vi "4Pi Dual DM Control.vi"(7 "Calling VI Ref":refnum<vi>) -> ()   [LabVIEW 2021]
uses:
  4Pi Dual DM - Controls/4Pi Dual DM - Mirror Modes.ctl
  4Pi Dual DM - Controls/DM Max Voltages.ctl
  <vilib>/Utility/miscctls.llb/LVPointTypeDef.ctl
  4Pi Dual DM - Controls/4Pi Dual DM - Mirror Order.ctl
  4Pi Dual DM - Controls/4Pi Dual DM - Standard Action.ctl
  <vilib>/Analysis/baseanly.llb/Mean (DBL).vi
  <vilib>/Utility/file.llb/Read Delimited Spreadsheet (DBL).vi
  <vilib>/Utility/file.llb/Write Delimited Spreadsheet (DBL).vi
  <vilib>/Analysis/NI_AALBase.lvlib
panel:
  in  "DM Max Voltages (V)":T1
  in  "Scan Modes":bool
  in  "Astig On/Off":bool
  in  "Load Astig":bool
  in  "Active Mirror":enum32{"Mirror 1", "Mirror 2"}(radio)
  in  "Clear Modes":bool
  in  "Mirror Modes":T2
  in  "Load Modes":bool
  in  "Save Modes":bool
  in  "Load Flat":bool
  in  "Apply Zero":bool
  in  "Load V Map":bool
  in  "Save V Map":bool
  in  "Apply Flat":bool
  in  "Center Bias":bool
  in  "Quit":bool
  out "Pixel Map (-1 to 1)":dbl[][](graph)
  # "Mode"
  # "Amount (nm)"
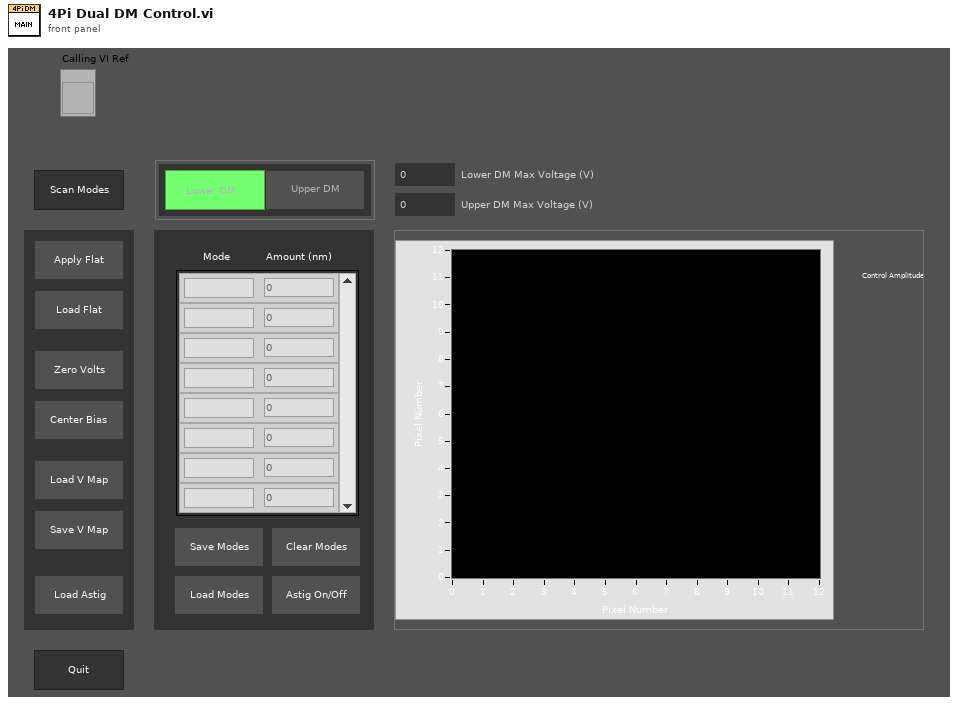
[diagram p1: front panel]
types:
  T1 = typedef "DM Max Voltages.ctl" = cluster{"Lower DM Max Voltage (V)":dbl, "Upper DM Max Voltage (V)":dbl}
  T2 = typedef "4Pi Dual DM - Mirror Modes.ctl" = cluster{"Mode":string, "Amplitude":dbl}[]
  T3 = typedef "4Pi Dual DM - Mirror Order.ctl" = cluster{"Flip Mirror Order":bool}
  T4 = enum16{"Always On", "Always Off", "Off While Running"}
  T5 = typedef "LVPointTypeDef.ctl" = cluster{"Horizontal":i16, "Vertical":i16}
  T6 = typedef "4Pi Dual DM - Standard Action.ctl" = enum16{"Read", "Write"}
  T7 = typedef "LVRectTypeDef.ctl" = cluster{"Left":i16, "Top":i16, "Right":i16, "Bottom":i16}
  T8 = typedef "LVBoundsTypeDef.ctl" = cluster{"Width":u32, "Height":u32}
  T9 = typedef "4Pi Dual DM - Mirror Modes DUAL.ctl" = cluster{"Mode":string, "Amplitude":dbl}[][]
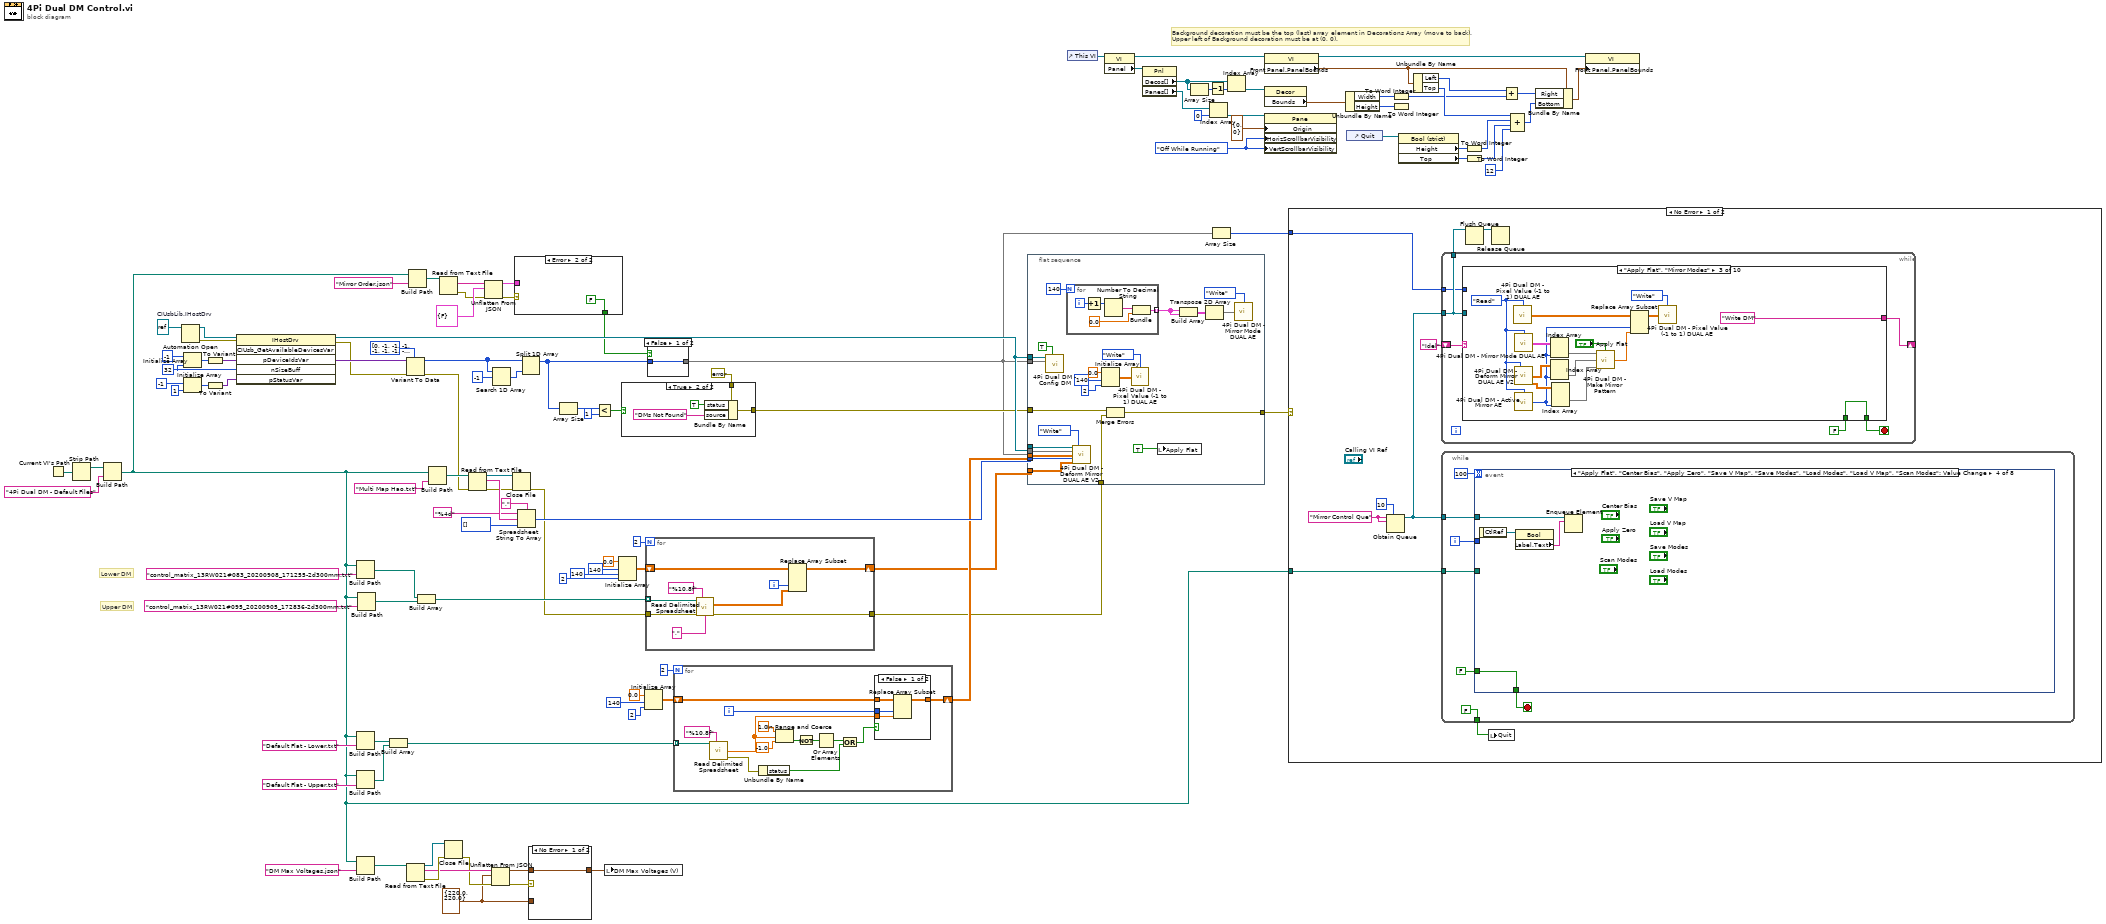
[diagram p0: block diagram]
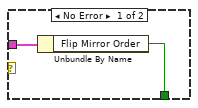
[diagram p2: hidden frame]
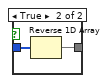
[diagram p4: hidden frame]
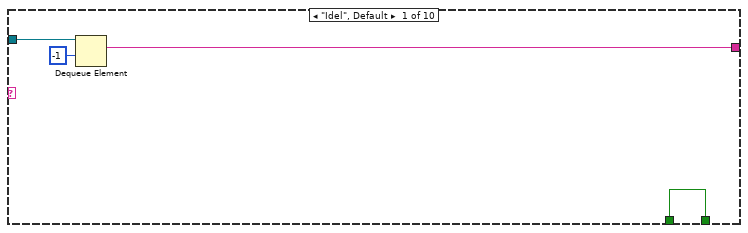
[diagram p5: hidden frame]
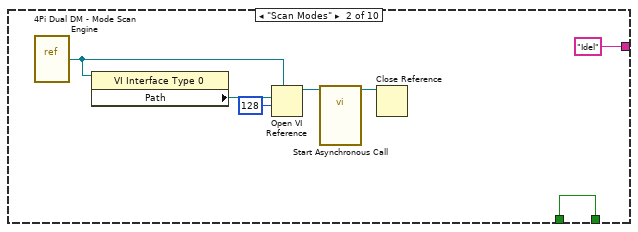
[diagram p6: hidden frame]
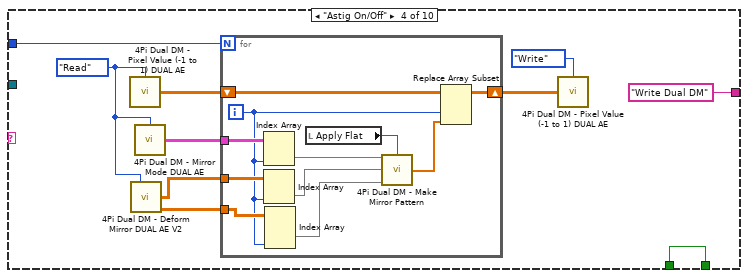
[diagram p7: hidden frame]
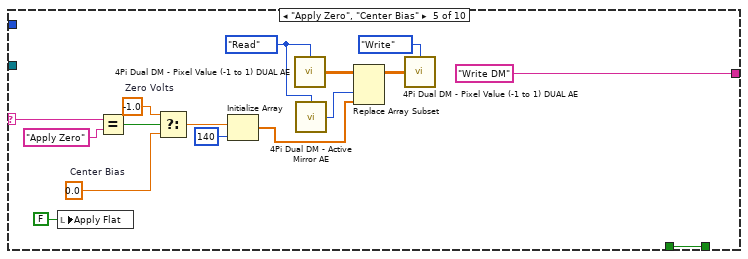
[diagram p8: hidden frame]
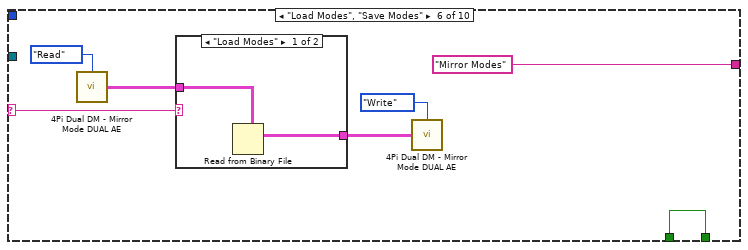
[diagram p9: hidden frame]
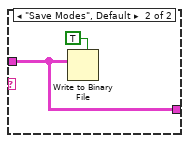
[diagram p10: hidden frame]
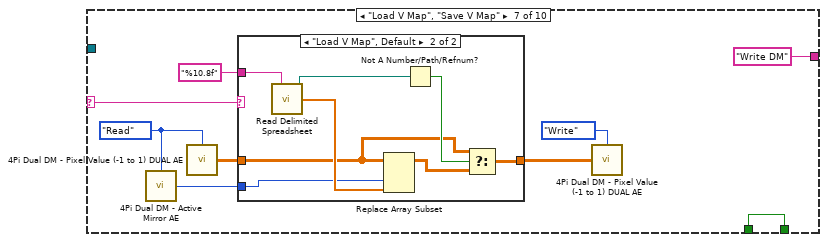
[diagram p11: hidden frame]
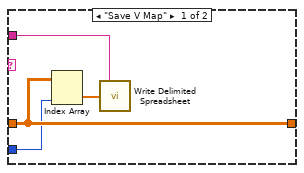
[diagram p12: hidden frame]
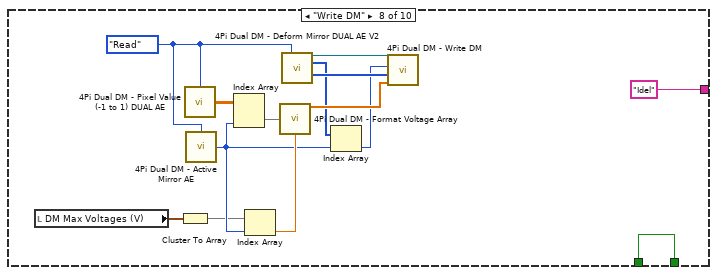
[diagram p13: hidden frame]
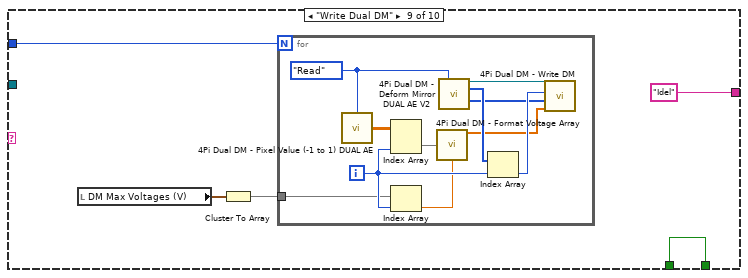
[diagram p14: hidden frame]
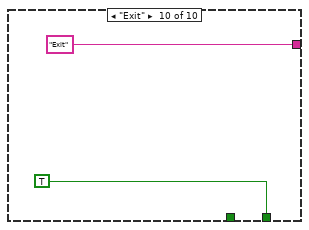
[diagram p15: hidden frame]
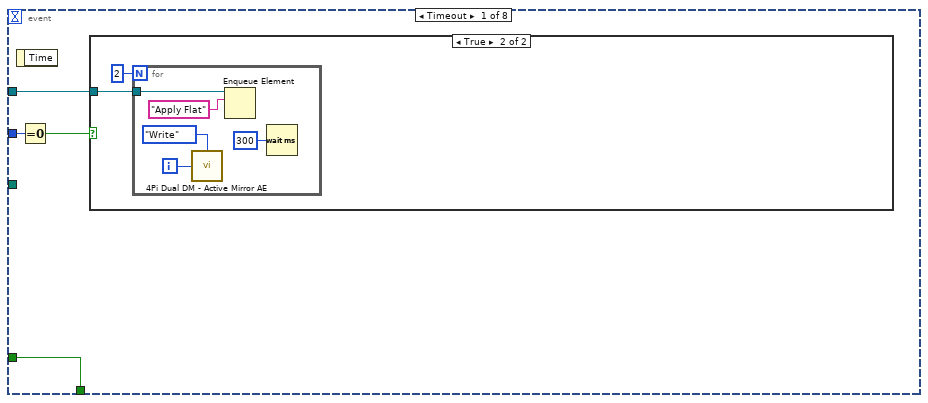
[diagram p16: hidden frame]
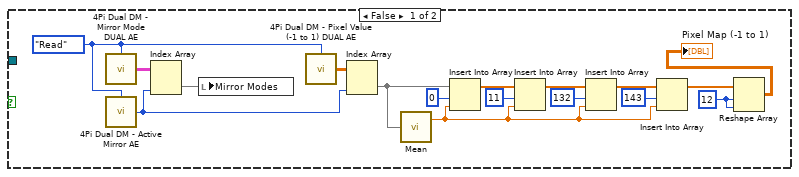
[diagram p17: hidden frame]
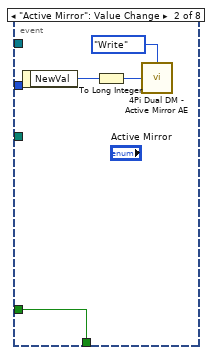
[diagram p18: hidden frame]
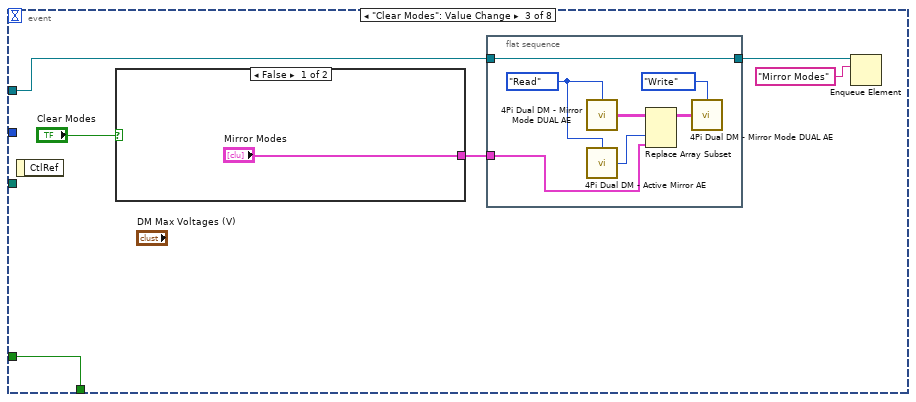
[diagram p19: hidden frame]
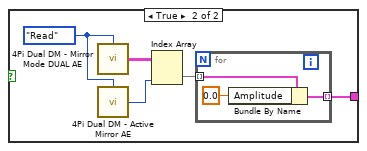
[diagram p20: hidden frame]
diagram:
  w21 = T1 {"Lower DM Max Voltage (V)"=220.0, "Upper DM Max Voltage (V)"=220.0} ("DM Max Voltages (V)")
  w79 = 32 ("dimension size")
  w70 = refnum<k7> refnum  # CIUsbLib.IHostDrv
  w96 = T4."Off While Running" ("Vertical Scrollbar Visibility")
  # "Upper DM"
  # "Lower DM"
  # "Background decoration must be the top (last) array element in Decorations Array (move to back).\nUpper left of Background decoration must be at (0, 0)."
  n1 = Current VI's Path() -> (path=w58:path)
  n2 = Strip Path(path=w58) -> (stripped path=w59:path)  [unwired: 1 out]
  n3 = Build Path(base path=w59, name or relative path="4Pi Dual DM - Default Files") -> (appended path=w10:path)
  n4 = Automation Open(Automation Refnum=w70) -> (Automation Refnum=w75:refnum<k7>, error out=w76:errorcluster)  [unwired: 1 in, 2 out]
  n5 = Initialize Array(-1 ("element"), w79) -> (w72:i32[])
  n6 = Initialize Array(-1 ("element"), 1 ("dimension size")) -> (w71:i32[])
  n7 = To Variant(anything=w72) -> (Variant=w73:variant)
  n8 = To Variant(anything=w71) -> (Variant=w78:variant)
  n9 = invoke class="IHostDrv" method="CIUsb_GetAvailableDevicesVar"(reference=w75, error in=w76, "pDeviceIdsVar"=w73, "nSizeBuff"=w79, "pStatusVar"=w78) -> (reference out=w37:refnum<k7>, error out=w54:errorcluster, "pDeviceIdsVar"=w84:variant)  [unwired: 1 in, 3 out]
  n10 = Build Path(base path=w10, name or relative path="Default Flat - Lower.txt") -> (appended path=w46:path)
  n11 = Build Path(base path=w10, name or relative path="Default Flat - Upper.txt") -> (appended path=w45:path)
  n12 = Build Path(base path=w10, name or relative path="DM Max Voltages.json") -> (appended path=w27:path)
  n13 = Build Path(base path=w10, name or relative path="control_matrix_13RW021#083_20200908_171255-2d300mm.txt") -> (appended path=w8:path)
  n14 = Build Path(base path=w10, name or relative path="control_matrix_13RW021#095_20200905_172836-2d300mm.txt") -> (appended path=w7:path)
  n15 = Build Array(w46, w45) -> (w44:path[])
  n16 = Variant To Data(error in=w54, type=i32[] [0, -1, -1, -1, -1, -1, -1, -1, -1, -1, -1, -1, -1, -1, -1, -1, -1, -1, -1, -1, -1, -1, -1, -1, -1, -1, -1, -1, -1, -1, -1, -1] ("pDeviceIDs"), Variant=w84) -> (data=w82:i32[], error out=w42:errorcluster)
  n17 = Read from Text File(file (use dialog)=w27) -> (refnum out=w26:refnum<file>, text=w24:string, error out=w25:errorcluster)  [unwired: 3 in, 1 out]
  n18 = Build Path(base path=w10, name or relative path="Mirror Order.json") -> (appended path=w34:path)
  n19 = Build Array(w8, w7) -> (w6:path[])
  n20 = Build Path(base path=w10, name or relative path="Multi Map Hao.txt") -> (appended path=w63:path)
  n21 = Read from Text File(file (use dialog)=w34) -> (text=w33:string, error out=w29:errorcluster)  [unwired: 3 in, 2 out]
  n22 = Close File(refnum=w26, error in=w25) -> (error out=w23:errorcluster)  [unwired: 1 out]
  n23 = Read from Text File(file (use dialog)=w63, error in=w42) -> (refnum out=w65:refnum<file>, text=w69:string, error out=w64:errorcluster)  [unwired: 3 out]
  n24 = Unflatten From JSON(JSON string=w33, type and defaults=T3 {"Flip Mirror Order"=FALSE} ("Mirror Order"), error in (no error)=w29) -> (value=w31:T3, error out=w17:errorcluster)  [unwired: 4 in]
  n25 = Unflatten From JSON(JSON string=w24, type and defaults=w21, error in (no error)=w23) -> (value=w20:T1, error out=w22:errorcluster)  [unwired: 4 in]
  n26 = Search 1D Array(1D array=w82, element=-1) -> (index of element=w81:i32)  [unwired: 1 in]
  n27 = Close File(refnum=w65, error in=w64) -> (error out=w4:errorcluster)  [unwired: 1 out]
  n28 = case shown="Error" w17 {
    tunnel: w31 -> [w115 _]
    tunnel: [w114 FALSE ("Flip Mirror Order")] -> w30
    frame No Error {
      n29 = Unbundle By Name(w115) -> ("Flip Mirror Order"=w114:bool)
    }
    frame Error {
    }
  }
  n30 = Spreadsheet String To Array(delimiter (Tab)=",", format string="%4d", spreadsheet string=w69, array type (2D Dbl)=i32[] []) -> (array=w61:i32[])
  n31 = Split 1D Array(array=w82, index=w81) -> (first subarray=w60:i32[])  [unwired: 1 out]
  n32 = case shown="No Error" w22 {
    tunnel: w21 -> [_ w118]
    tunnel: w20 -> [w117 _]
    tunnel: [w117 w118] -> w19
    frame No Error {
    }
    frame Error {
    }
  }
  n33 = Array Size(array=w60) -> (size(s)=w41:i32)
  n34 = Less?(x=w41, y=1) -> (x < y?=w39:bool)
  n35 = local write "DM Max Voltages (V)"(w19) -> ()
  n36 = Initialize Array(0.0 ("element"), 140 ("dimension size"), 140 ("dimension size"), 2 ("dimension size")) -> (w5:dbl[][][])
  n37 = case shown="True" w39 {
    tunnel: [w119 w121] -> w18
    tunnel: errorcluster {"status"=FALSE, "code"=0, "source"=""} ("error out") -> [w119 w120]
    frame False {
    }
    frame True {
      n38 = Bundle By Name(cluster=w120, "status"=TRUE, "source"="DMs Not Found" ("message")) -> (w121:errorcluster)
    }
  }
  n39 = Initialize Array(0.0 ("element"), 140 ("dimension size"), 2 ("dimension size")) -> (w49:dbl[][])
  n40 = for {
    N: 2 -> [_]
    tunnel: w6 -> [w130] mode=indexing
    shift-right: [w128] -> w1
    shift-left: w5 -> [w129]
    tunnel: w4 -> [w125]
    tunnel: [w124] -> w3
    i -> [w127]
    n41 = call-poly <vilib>:"Read Delimited Spreadsheet.vi"("file path (dialog if empty)"=w130, "format (%.3f)"="%10.8f", "error in (no error)"=w125, "delimiter (\\t)"="," ("delimiter (\\t)")) -> ("all rows"=w126:dbl[][], "error out"=w124:errorcluster)  [unwired: 6 in, 4 out]
    n42 = Replace Array Subset(array=w129, new element=w126, index (dim 2)=w127) -> (w128:dbl[][][])  [unwired: 2 in]
  }
  n43 = case shown="False" w30 {
    tunnel: w60 -> [w133 w135]
    tunnel: [w133 w134] -> w16
    frame False {
    }
    frame True {
      n44 = Reverse 1D Array(array=w135) -> (reversed array=w134:i32[])
    }
  }
  n45 = for {
    N: 2 -> [_]
    shift-right: [w146] -> w43
    shift-left: w49 -> [w149]
    tunnel: w44 -> [w140] mode=indexing
    i -> [w148]
    n46 = call-poly <vilib>:"Read Delimited Spreadsheet.vi"("file path (dialog if empty)"=w140, "format (%.3f)"="%10.8f") -> ("first row"=w141:dbl[], "error out"=w139:errorcluster)  [unwired: 8 in, 4 out]
    n47 = Unbundle By Name(w139) -> ("status"=w137:bool)
    n48 = In Range and Coerce(upper limit=1.0, x=w141, lower limit=-1.0) -> (In Range?=w143:bool[])  [unwired: 1 out]
    n49 = Not(x=w143) -> (.not. x?=w144:bool[])
    n50 = Or Array Elements(Boolean array=w144) -> (logical OR=w138:bool)
    n51 = Or(x=w138, y=w137) -> (x .or. y?=w136:bool)
    n52 = case shown="False" w136 {
      tunnel: w149 -> [w153 w154]
      tunnel: w148 -> [w152 _]
      tunnel: [w151 w154] -> w146
      tunnel: w141 -> [w150 _]
      frame False {
        n53 = Replace Array Subset(array=w153, new element=w150, index (col)=w152) -> (w151:dbl[][])  [unwired: 1 in]
      }
      frame True {
      }
    }
  }
  n54 = flat-sequence {
    tunnel: w37 -> [w176]
    tunnel: w61 -> [w174]
    tunnel: w16 -> [w173]
    tunnel: w43 -> [w172]
    tunnel: w18 -> [w171]
    tunnel: w3 -> [w170]
    tunnel: w37 -> [w169]
    tunnel: [w163] -> w36
    tunnel: w16 -> [w162]
    tunnel: w1 -> [w155]
    frame #0 {
      n55 = call "4Pi Dual DM - Config DM.vi"("High Voltage"=TRUE, "Dev IDs"=w173, "Automation Refnum in"=w169) -> ()  [unwired: 7 in, 2 out]
      n56 = for {
        N: 140 -> [_]
        tunnel: [w178] -> w159 mode=indexing
        i -> [w182]
        n57 = Increment(x=w182) -> (x+1=w181:i32)
        n58 = Number To Decimal String(number=w181) -> (decimal integer string=w180:string)  [unwired: 1 in]
        n59 = Bundle(w180, 0.0) -> (w178:cluster{string, dbl})  [unwired: 1 in]
      }
      n60 = call "4Pi Dual DM - Deform Mirror DUAL AE V2.vi"("Refnum In"=w176, "Action"=4Pi_Dual_DM_-_Standard_Action."Write", "IDs In"=w162, "Flat Files In"=w172, "Multi Map Data In"=w174, "Mode Matrix"=w155) -> ()  [unwired: 5 in, 5 out]
      n61 = Initialize Array(0.0 ("element"), 140 ("dimension size"), 2 ("dimension size")) -> (w167:dbl[][])
      n62 = Merge Errors(w171, w170) -> (w163:errorcluster)
      n63 = call "4Pi Dual DM - Pixel Value (-1 to 1) DUAL AE.vi"("Action"=4Pi_Dual_DM_-_Standard_Action."Write", "Pixel Value (-1 to 1)"=w167) -> ()  [unwired: 13 in, 1 out]
      n64 = local write "Apply Flat"(TRUE ("Apply Flat")) -> ()
      n65 = Build Array(w159, w159) -> (w160:cluster{string, dbl}[][])
      n66 = Transpose 2D Array(2D array=w160) -> (transposed array=w161:cluster{string, dbl}[][])
      n67 = call "4Pi Dual DM - Mirror Mode DUAL AE.vi"("Action"=4Pi_Dual_DM_-_Standard_Action."Write", "Mirror Modes In"=w161) -> ()  [unwired: 13 in, 1 out]
    }
  }
  n68 = control-ref of="This VI"() -> (w88:refnum<vi>)
  n69 = property class="VI"(reference=w88) -> (reference out=w97:refnum<vi>, "Panel"=w89:refnum<vi>)  [unwired: 1 in, 1 out]
  n70 = property class="Pnl"(reference=w89) -> ("Decos[]"=w87:refnum<vi>[], "Panes[]"=w93:refnum<vi>[])  [unwired: 1 in, 2 out]
  n71 = Array Size(array=w87) -> (size(s)=w85:i32)
  n72 = Decrement(x=w85) -> (x-1=w86:i32)
  n73 = Index Array(array=w93, index=0) -> (element=w92:refnum<vi>)
  n74 = Array Size(array=w16) -> (size(s)=w15:i32)
  n75 = Index Array(array=w87, index=w86) -> (element=w95:refnum<vi>)
  n76 = property class="VI"(reference=w97) -> (reference out=w99:refnum<vi>, "Front Panel.PanelBounds"=w100:T7)  [unwired: 1 in, 1 out]
  n77 = property class="Decor"(reference=w95) -> ("Bounds"=w98:T8)  [unwired: 1 in, 2 out]
  n78 = property class="Pane"(reference=w92, "Origin"=T5 {"Horizontal"=0, "Vertical"=0}, "HorizScrollbarVisibility"=w96, "VertScrollbarVisibility"=w96) -> ()  [unwired: 1 in, 2 out]
  n79 = case shown="No Error" w36 {
    tunnel: w10 -> [w184 _]
    tunnel: w15 -> [w183 _]
    frame No Error {
      w191 = "Mirror Control Que" ("name (unnamed)")
      n80 = Obtain Queue(max queue size (-1, unlimited)=10, name (unnamed)=w191, element data type=w191) -> (queue out=w186:refnum<queue>)  [unwired: 2 in, 2 out]
      n81 = while {
        tunnel: w186 -> [w193]
        shift-right: [w197] -> _
        shift-left: "Idel" ("name (unnamed)") -> [w196]
        tunnel: [w193] -> w189
        tunnel: w183 -> [w192]
        stop <- w195 stop-if-true
        n82 = case shown="\"Apply Flat\", \"Mirror Modes\"" w196 {
          selector: w196 -> [_ _ _ _ w256 w263 w279 _ _ _]
          tunnel: w193 -> [w201 _ _ _ _ _ _ _ _ _]
          tunnel: [w199 "Idel" ("name (unnamed)") "Write DM" ("name (unnamed)") "Write Dual DM" ("name (unnamed)") "Write DM" ("name (unnamed)") "Mirror Modes" ("name (unnamed)") "Write DM" ("name (unnamed)") "Idel" ("name (unnamed)") "Idel" ("name (unnamed)") "Exit" ("name (unnamed)")] -> w197
          tunnel: [w198 w208 w222 w232 w260 w267 w280 w306 w311 TRUE] -> w195
          tunnel: FALSE -> [w198 w208 w222 w232 w260 w267 w280 w306 w311 _]
          tunnel: w192 -> [_ _ _ w226 _ _ _ _ w307 _]
          frame "Idel", Default {
            n83 = Dequeue Element(queue=w201, timeout in ms (-1)=-1) -> (element=w199:string)  [unwired: 1 in, 3 out]
          }
          frame "Scan Modes" {
            n84 = vi-ref "4Pi Dual DM - Mode Scan Engine.vi"() -> (w202:refnum<vi>)
            n85 = property class="VI Interface Type 0"(reference=w202) -> ("Path"=w203:path)  [unwired: 1 in, 2 out]
            n86 = Open VI Reference(type specifier VI Refnum (for type only)=w202, vi path=w203, options=128) -> (vi reference=w205:refnum<vi>)  [unwired: 3 in, 1 out]
            n87 = call-by-ref "Start Asynchronous Call"(reference=w205) -> (reference out=w206:refnum<vi>)  [unwired: 17 in, 1 out]
            n88 = Close Reference(reference=w206) -> ()  [unwired: 1 in, 1 out]
          }
          frame "Apply Flat", "Mirror Modes" {
            w218 = 4Pi_Dual_DM_-_Standard_Action."Read" ("Action")
            n89 = call "4Pi Dual DM - Pixel Value (-1 to 1) DUAL AE.vi"("Action"=w218) -> ("Pixel Value (-1 to 1) Out"=w219:dbl[][])  [unwired: 14 in]
            n90 = call "4Pi Dual DM - Mirror Mode DUAL AE.vi"("Action"=w218) -> ("Mirror Modes Out"=w215:T9)  [unwired: 14 in]
            n91 = call "4Pi Dual DM - Deform Mirror DUAL AE V2.vi"("Action"=w218) -> ("Flat Files Out"=w213:dbl[][], "Mode Matrix Out"=w211:dbl[][][])  [unwired: 10 in, 3 out]
            n92 = call "4Pi Dual DM - Active Mirror AE.vi"("Action"=w218) -> ("Active Mirror"=w210:i32)  [unwired: 14 in]
            n93 = Index Array(array=w215, index (col)=w210) -> (element=w216:cluster{"Mode":string, "Amplitude":dbl}[])  [unwired: 1 in]
            n94 = Index Array(array=w213, index (col)=w210) -> (element=w214:dbl[])  [unwired: 1 in]
            n95 = Index Array(array=w211, index (dim 2)=w210) -> (element=w209:dbl[][])  [unwired: 2 in]
            n96 = call "4Pi Dual DM - Make Mirror Pattern.vi"("Mirror Modes In"=w216, "Flat On?"="Apply Flat", "Flat File In"=w214, "Mirror Modes Array"=w209) -> ("Pixel Value U (-1 to 1)"=w220:dbl[])  [unwired: 11 in]
            n97 = Replace Array Subset(array=w219, new element=w220, index (col)=w210) -> (w221:dbl[][])  [unwired: 1 in]
            n98 = call "4Pi Dual DM - Pixel Value (-1 to 1) DUAL AE.vi"("Action"=4Pi_Dual_DM_-_Standard_Action."Write", "Pixel Value (-1 to 1)"=w221) -> ()  [unwired: 13 in, 1 out]
          }
          frame "Astig On/Off" {
            w231 = 4Pi_Dual_DM_-_Standard_Action."Read" ("Action")
            n99 = call "4Pi Dual DM - Pixel Value (-1 to 1) DUAL AE.vi"("Action"=w231) -> ("Pixel Value (-1 to 1) Out"=w230:dbl[][])  [unwired: 14 in]
            n100 = call "4Pi Dual DM - Deform Mirror DUAL AE V2.vi"("Action"=w231) -> ("Flat Files Out"=w228:dbl[][], "Mode Matrix Out"=w227:dbl[][][])  [unwired: 10 in, 3 out]
            n101 = call "4Pi Dual DM - Mirror Mode DUAL AE.vi"("Action"=w231) -> ("Mirror Modes Out"=w229:T9)  [unwired: 14 in]
            n102 = for {
              N: w226 -> [_]
              tunnel: w229 -> [w239]
              tunnel: w228 -> [w238]
              tunnel: w227 -> [w236]
              shift-right: [w237] -> w224
              shift-left: w230 -> [w240]
              i -> [w235]
              n103 = Index Array(array=w239, index (col)=w235) -> (element=w243:cluster{"Mode":string, "Amplitude":dbl}[])  [unwired: 1 in]
              n104 = Index Array(array=w238, index (col)=w235) -> (element=w244:dbl[])  [unwired: 1 in]
              n105 = Index Array(array=w236, index (dim 2)=w235) -> (element=w234:dbl[][])  [unwired: 2 in]
              n106 = local read "Apply Flat"() -> (w241:bool)
              n107 = call "4Pi Dual DM - Make Mirror Pattern.vi"("Mirror Modes In"=w243, "Flat On?"=w241, "Flat File In"=w244, "Mirror Modes Array"=w234) -> ("Pixel Value U (-1 to 1)"=w242:dbl[])  [unwired: 11 in]
              n108 = Replace Array Subset(array=w240, new element=w242, index (col)=w235) -> (w237:dbl[][])  [unwired: 1 in]
            }
            n109 = call "4Pi Dual DM - Pixel Value (-1 to 1) DUAL AE.vi"("Action"=4Pi_Dual_DM_-_Standard_Action."Write", "Pixel Value (-1 to 1)"=w224) -> ()  [unwired: 13 in, 1 out]
          }
          frame "Apply Zero", "Center Bias" {
            w248 = 4Pi_Dual_DM_-_Standard_Action."Read" ("Action")
            w252 = -1.0  # Zero Volts
            w254 = 0.0  # Center Bias
            n110 = local write "Apply Flat"(FALSE ("Apply Flat")) -> ()
            n111 = Equal?(x=w256, y="Apply Zero") -> (x = y?=w255:bool)
            n112 = Select(t=w252, s=w255, f=w254) -> (s? t:f=w253:dbl)
            n113 = Initialize Array(w253, 140 ("dimension size")) -> (w245:dbl[])
            n114 = call "4Pi Dual DM - Pixel Value (-1 to 1) DUAL AE.vi"("Action"=w248) -> ("Pixel Value (-1 to 1) Out"=w246:dbl[][])  [unwired: 14 in]
            n115 = call "4Pi Dual DM - Active Mirror AE.vi"("Action"=w248) -> ("Active Mirror"=w247:i32)  [unwired: 14 in]
            n116 = Replace Array Subset(array=w246, new element=w245, index (col)=w247) -> (w250:dbl[][])  [unwired: 1 in]
            n117 = call "4Pi Dual DM - Pixel Value (-1 to 1) DUAL AE.vi"("Action"=4Pi_Dual_DM_-_Standard_Action."Write", "Pixel Value (-1 to 1)"=w250) -> ()  [unwired: 13 in, 1 out]
          }
          frame "Load Modes", "Save Modes" {
            n118 = call "4Pi Dual DM - Mirror Mode DUAL AE.vi"("Action"=4Pi_Dual_DM_-_Standard_Action."Read") -> ("Mirror Modes Out"=w262:T9)  [unwired: 14 in]
            n119 = case shown="\"Load Modes\"" w263 {
              tunnel: w262 -> [w269 w270]
              tunnel: [w268 w270] -> w261
              frame "Load Modes" {
                n120 = Read from Binary File(5:w269) -> (2:w268:T9)  [unwired: 5 in, 3 out]
              }
              frame "Save Modes", Default {
                n121 = Write to Binary File(data=w270, 5:TRUE ("prepend array or string size? (T)")) -> ()  [unwired: 4 in, 3 out]
              }
            }
            n122 = call "4Pi Dual DM - Mirror Mode DUAL AE.vi"("Action"=4Pi_Dual_DM_-_Standard_Action."Write", "Mirror Modes In"=w261) -> ()  [unwired: 13 in, 1 out]
          }
          frame "Load V Map", "Save V Map" {
            w273 = 4Pi_Dual_DM_-_Standard_Action."Read" ("Action")
            n123 = call "4Pi Dual DM - Active Mirror AE.vi"("Action"=w273) -> ("Active Mirror"=w272:i32)  [unwired: 14 in]
            n124 = call "4Pi Dual DM - Pixel Value (-1 to 1) DUAL AE.vi"("Action"=w273) -> ("Pixel Value (-1 to 1) Out"=w277:dbl[][])  [unwired: 14 in]
            n125 = case shown="\"Load V Map\", Default" w279 {
              tunnel: w277 -> [w283 w285]
              tunnel: "%10.8f" -> [w284 w292]
              tunnel: [w283 w289] -> w274
              tunnel: w272 -> [w281 w286]
              frame "Save V Map" {
                n126 = Index Array(array=w283, index (col)=w281) -> (element=w282:dbl[])  [unwired: 1 in]
                n127 = call-poly <vilib>:"Write Delimited Spreadsheet.vi"("format (%.3f)"=w284, "1D data"=w282) -> ()  [unwired: 12 in, 2 out]
              }
              frame "Load V Map", Default {
                n128 = call-poly <vilib>:"Read Delimited Spreadsheet.vi"("format (%.3f)"=w292) -> ("new file path (Not A Path if cancelled)"=w291:path, "first row"=w287:dbl[])  [unwired: 9 in, 4 out]
                n129 = Replace Array Subset(array=w285, new element=w287, index (col)=w286) -> (w288:dbl[][])  [unwired: 1 in]
                n130 = Not A Number/Path/Refnum?(number/path/refnum=w291) -> (NaN/Path/Refnum?=w290:bool)
                n131 = Select(t=w285, s=w290, f=w288) -> (s? t:f=w289:dbl[][])
              }
            }
            n132 = call "4Pi Dual DM - Pixel Value (-1 to 1) DUAL AE.vi"("Action"=4Pi_Dual_DM_-_Standard_Action."Write", "Pixel Value (-1 to 1)"=w274) -> ()  [unwired: 13 in, 1 out]
          }
          frame "Write DM" {
            w299 = 4Pi_Dual_DM_-_Standard_Action."Read" ("Action")
            n133 = local read "DM Max Voltages (V)"() -> (w294:T1)
            n134 = Cluster To Array(cluster=w294) -> (array=w293:dbl[])
            n135 = call "4Pi Dual DM - Pixel Value (-1 to 1) DUAL AE.vi"("Action"=w299) -> ("Pixel Value (-1 to 1) Out"=w301:dbl[][])  [unwired: 14 in]
            n136 = call "4Pi Dual DM - Active Mirror AE.vi"("Action"=w299) -> ("Active Mirror"=w295:i32)  [unwired: 14 in]
            n137 = Index Array(array=w301, index (col)=w295) -> (element=w300:dbl[])  [unwired: 1 in]
            n138 = Index Array(array=w293, index=w295) -> (element=w296:dbl)
            n139 = call "4Pi Dual DM - Format Voltage Array.vi"("Pixel Level (-1 to 1)"=w300, "Max DM Voltage"=w296) -> ("Voltage Array (Volts)"=w302:dbl[])  [unwired: 12 in, 1 out]
            n140 = call "4Pi Dual DM - Deform Mirror DUAL AE V2.vi"("Action"=w299) -> ("Refnum Out"=w304:refnum<k7>, "IDs Out"=w298:i32[], "Multi Map Data Out"=w303:i32[])  [unwired: 10 in, 2 out]
            n141 = Index Array(array=w298, index=w295) -> (element=w297:i32)
            n142 = call "4Pi Dual DM - Write DM.vi"("reference in"=w304, "nDevId"=w297, "MultiDM  Mapping"=w303, "Voltage Array in"=w302) -> ()  [unwired: 2 in, 2 out]
          }
          frame "Write Dual DM" {
            n143 = local read "DM Max Voltages (V)"() -> (w309:T1)
            n144 = Cluster To Array(cluster=w309) -> (array=w308:dbl[])
            n145 = for {
              N: w307 -> [_]
              tunnel: w308 -> [w313]
              i -> [w314]
              w320 = 4Pi_Dual_DM_-_Standard_Action."Read" ("Action")
              n146 = call "4Pi Dual DM - Pixel Value (-1 to 1) DUAL AE.vi"("Action"=w320) -> ("Pixel Value (-1 to 1) Out"=w318:dbl[][])  [unwired: 14 in]
              n147 = Index Array(array=w318, index (col)=w314) -> (element=w319:dbl[])  [unwired: 1 in]
              n148 = Index Array(array=w313, index=w314) -> (element=w312:dbl)
              n149 = call "4Pi Dual DM - Format Voltage Array.vi"("Pixel Level (-1 to 1)"=w319, "Max DM Voltage"=w312) -> ("Voltage Array (Volts)"=w317:dbl[])  [unwired: 12 in, 1 out]
              n150 = call "4Pi Dual DM - Deform Mirror DUAL AE V2.vi"("Action"=w320) -> ("Refnum Out"=w315:refnum<k7>, "IDs Out"=w321:i32[], "Multi Map Data Out"=w316:i32[])  [unwired: 10 in, 2 out]
              n151 = Index Array(array=w321, index=w314) -> (element=w322:i32)
              n152 = call "4Pi Dual DM - Write DM.vi"("reference in"=w315, "nDevId"=w322, "MultiDM  Mapping"=w316, "Voltage Array in"=w317) -> ()  [unwired: 2 in, 2 out]
            }
          }
          frame "Exit" {
          }
        }
      }
      n153 = while {
        tunnel: w186 -> [w327]
        tunnel: [FALSE] -> w185
        tunnel: w184 -> [w325]
        i -> [w328]
        stop <- w331 stop-if-true
        n154 = event shown="[3] \"Apply Flat\", \"Center Bias\", \"Apply Zero\", \"Save V Map\", \"Save Modes\", \"Load Modes\", \"Load V Map\", \"Scan Modes\": Value Change" {
          selector: _ -> [_ _ _ _ _ _ _ _]
          dyn-events: _ -> [_ _ _ _ _ _ _ _]
          timeout: 100 -> [_ _ _ _ _ _ _ _]
          tunnel: [w335 w363 w369 w389 w394 w418 w427 w456] -> w331
          tunnel: FALSE -> [w335 w363 w369 w389 w394 w418 w427 _]
          tunnel: w328 -> [w334 _ _ _ _ _ _ _]
          tunnel: w327 -> [w332 _ w368 w388 _ _ w424 w454]
          tunnel: w325 -> [_ _ _ _ w393 w416 _ _]
          event Timeout {
            n155 = event-data() -> ()  [unwired: 1 in, 1 out]
            n156 = Equal To 0?(x=w334) -> (x = 0?=w333:bool)
            n157 = case shown="True" w333 {
              tunnel: w332 -> [_ w354]
              frame False {
                w348 = 12 ("dimension size")
                w349 = 4Pi_Dual_DM_-_Standard_Action."Read" ("Action")
                n158 = call "4Pi Dual DM - Mirror Mode DUAL AE.vi"("Action"=w349) -> ("Mirror Modes Out"=w336:T9)  [unwired: 14 in]
                n159 = call "4Pi Dual DM - Active Mirror AE.vi"("Action"=w349) -> ("Active Mirror"=w351:i32)  [unwired: 14 in]
                n160 = Index Array(array=w336, index (col)=w351) -> (element=w337:cluster{"Mode":string, "Amplitude":dbl}[])  [unwired: 1 in]
                n161 = local write "Mirror Modes"(w337) -> ()
                n162 = call "4Pi Dual DM - Pixel Value (-1 to 1) DUAL AE.vi"("Action"=w349) -> ("Pixel Value (-1 to 1) Out"=w350:dbl[][])  [unwired: 14 in]
                n163 = Index Array(array=w350, index (col)=w351) -> (element=w352:dbl[])  [unwired: 1 in]
                n164 = call-poly <vilib>:"Mean.vi"("X"=w352) -> ("mean"=w346:dbl)  [unwired: 1 out]
                n165 = Insert Into Array(array=w352, index=0, new element=w346) -> (w341:dbl[])
                n166 = Insert Into Array(array=w341, index=11, new element=w346) -> (w343:dbl[])
                n167 = Insert Into Array(array=w343, index=132, new element=w346) -> (w345:dbl[])
                n168 = Insert Into Array(array=w345, index=143, new element=w346) -> (w338:dbl[])
                n169 = Reshape Array(w338, w348, w348) -> (→"Pixel Map (-1 to 1)":dbl[][])
              }
              frame True {
                n170 = for {
                  N: 2 -> [_]
                  tunnel: w354 -> [w359]
                  i -> [w355]
                  n171 = call "4Pi Dual DM - Active Mirror AE.vi"("Action"=4Pi_Dual_DM_-_Standard_Action."Write", "Active Mirror In"=w355) -> ()  [unwired: 13 in, 1 out]
                  n172 = Enqueue Element(queue=w359, element="Apply Flat") -> ()  [unwired: 2 in, 3 out]
                  n173 = Wait (ms)(milliseconds to wait=u32 300) -> ()  [unwired: 1 out]
                }
              }
            }
          }
          event "Active Mirror": Value Change {
            n174 = event-data() -> ("NewVal"=w362:enum32{"Mirror 1", "Mirror 2"})  [unwired: 1 in]
            n175 = To Long Integer(number=w362) -> (32bit integer=w361:i32)
            n176 = call "4Pi Dual DM - Active Mirror AE.vi"("Action"=4Pi_Dual_DM_-_Standard_Action."Write", "Active Mirror In"=w361) -> ()  [unwired: 13 in, 1 out]
          }
          event "Clear Modes": Value Change {
            n177 = event-data() -> ()  [unwired: 1 in, 1 out]
            n178 = case shown="False" "Clear Modes" {
              tunnel: ["Mirror Modes" w371] -> w364
              frame False {
              }
              frame True {
                w374 = 4Pi_Dual_DM_-_Standard_Action."Read" ("Action")
                n179 = call "4Pi Dual DM - Mirror Mode DUAL AE.vi"("Action"=w374) -> ("Mirror Modes Out"=w373:T9)  [unwired: 14 in]
                n180 = call "4Pi Dual DM - Active Mirror AE.vi"("Action"=w374) -> ("Active Mirror"=w375:i32)  [unwired: 14 in]
                n181 = Index Array(array=w373, index (col)=w375) -> (element=w372:cluster{"Mode":string, "Amplitude":dbl}[])  [unwired: 1 in]
                n182 = for {
                  tunnel: w372 -> [w378] mode=indexing
                  tunnel: [w376] -> w371 mode=indexing
                  n183 = Bundle By Name(cluster=w378, "Amplitude"=0.0) -> (w376:cluster{"Mode":string, "Amplitude":dbl})
                }
              }
            }
            n184 = flat-sequence {
              tunnel: w364 -> [w379]
              tunnel: w368 -> [w385]
              tunnel: [w385] -> w366
              frame #0 {
                w382 = 4Pi_Dual_DM_-_Standard_Action."Read" ("Action")
                n185 = call "4Pi Dual DM - Mirror Mode DUAL AE.vi"("Action"=w382) -> ("Mirror Modes Out"=w381:T9)  [unwired: 14 in]
                n186 = call "4Pi Dual DM - Active Mirror AE.vi"("Action"=w382) -> ("Active Mirror"=w383:i32)  [unwired: 14 in]
                n187 = Replace Array Subset(array=w381, new element=w379, index (col)=w383) -> (w384:T9)  [unwired: 1 in]
                n188 = call "4Pi Dual DM - Mirror Mode DUAL AE.vi"("Action"=4Pi_Dual_DM_-_Standard_Action."Write", "Mirror Modes In"=w384) -> ()  [unwired: 13 in, 1 out]
              }
            }
            n189 = Enqueue Element(queue=w366, element="Mirror Modes") -> ()  [unwired: 2 in, 3 out]
          }
          event "Apply Flat", "Center Bias", "Apply Zero", "Save V Map", "Save Modes", "Load Modes", "Load V Map", "Scan Modes": Value Change {
            n190 = event-data() -> ("CtlRef"=w387:refnum<vi>)  [unwired: 1 in]
            n191 = property class="Bool"(reference=w387) -> ("Label.Text"=w386:string)  [unwired: 1 in, 2 out]
            n192 = Enqueue Element(queue=w388, element=w386) -> ()  [unwired: 2 in, 3 out]
          }
          event "Load Flat": Value Change {
            n193 = event-data() -> ()  [unwired: 1 in, 1 out]
            n194 = call "File Dialog"("start path"=w393, "prompt"="Select Flat File") -> ("selected path"=w390:path, "error out"=w391:errorcluster)  [unwired: 10 in, 2 out]
            n195 = case shown="No Error" w391 {
              tunnel: w390 -> [w395 _]
              frame No Error {
                w402 = 4Pi_Dual_DM_-_Standard_Action."Read" ("Action")
                n196 = call-poly <vilib>:"Read Delimited Spreadsheet.vi"("file path (dialog if empty)"=w395, "format (%.3f)"="%10.8f") -> ("first row"=w411:dbl[])  [unwired: 8 in, 5 out]
                n197 = In Range and Coerce(upper limit=1.0, x=w411, lower limit=-1.0) -> (coerced(x)=w396:dbl[], In Range?=w408:bool[])
                n198 = call "4Pi Dual DM - Deform Mirror DUAL AE V2.vi"("Action"=w402) -> ("Refnum Out"=w397:refnum<k7>, "IDs Out"=w398:i32[], "Flat Files Out"=w403:dbl[][], "Multi Map Data Out"=w399:i32[], "Mode Matrix Out"=w400:dbl[][][])  [unwired: 10 in]
                n199 = call "4Pi Dual DM - Active Mirror AE.vi"("Action"=w402) -> ("Active Mirror"=w405:i32)  [unwired: 14 in]
                n200 = Not(x=w408) -> (.not. x?=w407:bool[])
                n201 = Replace Array Subset(array=w403, new element=w396, index (col)=w405) -> (w404:dbl[][])  [unwired: 1 in]
                n202 = Or Array Elements(Boolean array=w407) -> (logical OR=w406:bool)
                n203 = call "4Pi Dual DM - Deform Mirror DUAL AE V2.vi"("Refnum In"=w397, "Action"=4Pi_Dual_DM_-_Standard_Action."Write", "IDs In"=w398, "Flat Files In"=w404, "Multi Map Data In"=w399, "Mode Matrix"=w400) -> ()  [unwired: 5 in, 5 out]
                n204 = case shown="True" w406 {
                  frame False {
                  }
                  frame True {
                    n205 = One Button Dialog(message="Flat File Out of Range [-1, 1]") -> ()  [unwired: 1 in, 1 out]
                  }
                }
              }
              frame Error {
              }
            }
          }
          event "Load Astig": Value Change {
            n206 = event-data() -> ()  [unwired: 1 in, 1 out]
            n207 = call "File Dialog2"("start path"=w416, "prompt"="Select Astigmatism File") -> ("selected path"=w414:path, "error out"=w415:errorcluster)  [unwired: 10 in, 2 out]
            n208 = case shown="No Error" w415 {
              tunnel: w414 -> [w419 _]
              frame No Error {
                n209 = call "4Pi Dual DM - Astig Modes AE.vi"("Action"=4Pi_Dual_DM_-_Standard_Action."Read") -> ("Mirror Modes Out"=w423:T9)  [unwired: 14 in]
                n210 = Read from Binary File(5:w423, 11:w419) -> (2:w420:T9)  [unwired: 4 in, 3 out]
                n211 = call "4Pi Dual DM - Astig Modes AE.vi"("Action"=4Pi_Dual_DM_-_Standard_Action."Write", "Mirror Modes In"=w420) -> ()  [unwired: 13 in, 1 out]
              }
              frame Error {
              }
            }
          }
          event "Astig On/Off": Value Change {
            n212 = event-data() -> ()  [unwired: 1 in, 1 out]
            n213 = case shown="True" "Astig On/Off" {
              tunnel: [w432 w444] -> w425
              frame False {
                n214 = for {
                  N: 2 -> [_]
                  tunnel: [w435] -> w433 mode=indexing
                  i -> [w436]
                  n215 = call "4Pi Dual DM - Mirror Mode DUAL AE.vi"("Action"=4Pi_Dual_DM_-_Standard_Action."Read") -> ("Mirror Modes Out"=w438:T9)  [unwired: 14 in]
                  n216 = Index Array(array=w438, index (col)=w436) -> (element=w439:cluster{"Mode":string, "Amplitude":dbl}[])  [unwired: 1 in]
                  n217 = for {
                    tunnel: w439 -> [w442] mode=indexing
                    tunnel: [w440] -> w435 mode=indexing
                    n218 = Bundle By Name(cluster=w442, "Amplitude"=0.0) -> (w440:cluster{"Mode":string, "Amplitude":dbl})
                  }
                }
                n219 = Transpose 2D Array(2D array=w433) -> (transposed array=w432:cluster{"Mode":string, "Amplitude":dbl}[][])
              }
              frame True {
                n220 = call "4Pi Dual DM - Astig Modes AE.vi"("Action"=4Pi_Dual_DM_-_Standard_Action."Read") -> ("Mirror Modes Out"=w444:T9)  [unwired: 14 in]
              }
            }
            n221 = flat-sequence {
              tunnel: w425 -> [w429]
              tunnel: w424 -> [w430]
              frame #0 {
                n222 = call "4Pi Dual DM - Mirror Mode DUAL AE.vi"("Action"=4Pi_Dual_DM_-_Standard_Action."Write", "Mirror Modes In"=w429) -> ()  [unwired: 13 in, 1 out]
              }
              frame #1 {
                n223 = Enqueue Element(queue=w430, element="Astig On/Off") -> ()  [unwired: 2 in, 3 out]
              }
            }
          }
          event "Quit": Value Change {
            n224 = event-data() -> ("NewVal"=w456:bool)  [unwired: 1 in]
            n225 = for {
              N: 2 -> [_]
              tunnel: w454 -> [w462]
              tunnel: [w457] -> w445
              i -> [w458]
              n226 = call "4Pi Dual DM - Active Mirror AE.vi"("Action"=4Pi_Dual_DM_-_Standard_Action."Write", "Active Mirror In"=w458) -> ()  [unwired: 13 in, 1 out]
              n227 = Enqueue Element(queue=w462, element="Apply Zero") -> (queue out=w457:refnum<queue>)  [unwired: 2 in, 2 out]
              n228 = Wait (ms)(milliseconds to wait=u32 300) -> ()  [unwired: 1 out]
            }
            n229 = Enqueue Element(queue=w445, element="Exit") -> (error out=w449:errorcluster)  [unwired: 2 in, 2 out]
            n230 = call "4Pi Dual DM - Deform Mirror DUAL AE V2.vi"("Action"=4Pi_Dual_DM_-_Standard_Action."Read") -> ("Refnum Out"=w452:refnum<k7>, "IDs Out"=w447:i32[])  [unwired: 10 in, 3 out]
            n231 = call "4Pi Dual DM - Config DM.vi"("High Voltage"=FALSE, "error in (no error)"=w449, "Dev IDs"=w447, "Automation Refnum in"=w452) -> ("error out"=w448:errorcluster, "Automation Refnum out"=w451:refnum<k7>)  [unwired: 6 in]
            n232 = Close Reference(reference=w451, error in (no error)=w448) -> ()  [unwired: 1 out]
          }
        }
      }
      n233 = Flush Queue(queue=w189) -> (queue out=w188:refnum<queue>)  [unwired: 1 in, 2 out]
      n234 = local write "Quit"(w185) -> ()
      n235 = Release Queue(queue=w188) -> ()  [unwired: 2 in, 3 out]
    }
    frame Error {
      n236 = One Button Dialog(message="DMs not found.") -> ()  [unwired: 1 in, 1 out]
    }
  }
  n237 = Unbundle By Name(w98) -> ("Width"=w103:u32, "Height"=w106:u32)
  n238 = control-ref of="Quit"() -> (w90:refnum<vi>)
  n239 = To Word Integer(number=w103) -> (16bit integer=w105:i16)
  n240 = To Word Integer(number=w106) -> ()  [unwired: 1 out]
  n241 = property class="Bool (strict)"(reference=w90) -> ("Height"=w108:u32, "Top"=w109:i32)  [unwired: 1 in, 2 out]
  n242 = Unbundle By Name(w100) -> ("Left"=w102:i16, "Top"=w113:i16)
  n243 = To Word Integer(number=w108) -> (16bit integer=w111:i16)
  n244 = To Word Integer(number=w109) -> (16bit integer=w112:i16)
  n245 = Add(x=w102, y=w105) -> (x+y=w104:i16)
  n246 = Compound Arithmetic op=ADD(w113, w111, w112, i16 12 ("y")) -> (w107:i16)
  n247 = Bundle By Name(cluster=w100, "Right"=w104, "Bottom"=w107) -> (w101:T7)
  n248 = property class="VI"(reference=w99, "Front Panel.PanelBounds"=w101) -> ()  [unwired: 1 in, 2 out]
